vi "Module Init.vi"(8 "error in (no error)":errorcluster, 11 "DAQmxAO in":refnum<class "DAQmxAO.lvclass">) -> (0 "error out":errorcluster, 3 "DAQmxAO out":refnum<class "DAQmxAO.lvclass">)   [LabVIEW 2020, in "VolatusDAQ.lvlib" / "DAQmxAO.lvclass"]
uses:
  DAQmxAO.lvclass
  C:/dev/lv20CE/relink/lv-volatus/Volatus/Module/Module.lvclass
  Volatus/Message Registration.ctl
  VolatusData/DataProc Options.ctl
  DAQmxAO.lvclass/DAQmxAO.ctl
  Volatus/Module/Module.lvclass/Module.ctl
  Volatus/MessageQ/MessageQ.lvclass/MessageQ.ctl
  Volatus/Module/Self Q.vi
  Volatus/MessageQ/Send.vi
  VolatusDAQ.lvlib
  VolatusData/Data Processor Module/Data Processor Module.lvclass
  Volatus/Module/Module.lvclass
  Volatus/Volatus.lvlib
  VolatusData/VolatusData.lvlib
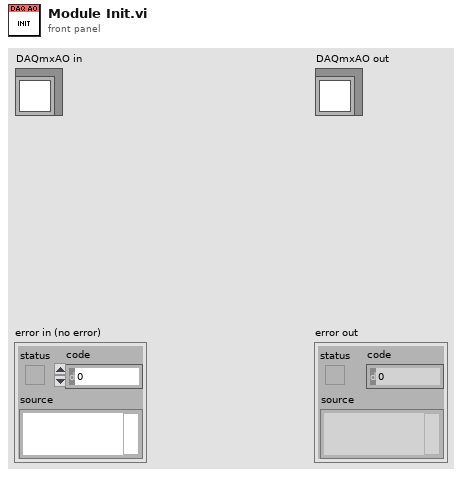
[diagram p1: front panel]
types:
  T1 = typedef "VolatusData.lvlib/DataProc Options.ctl" = cluster{"Ignore Scaling":bool}
  T2 = typedef "Volatus.lvlib/Message Registration.ctl" = cluster{"Message Type":string, "Message ID":string}
  T3 = typedef "VolatusDAQConfig.lvlib/Sampling Config.ctl" = cluster{"Rate":dbl, "Chunk Size":i32}
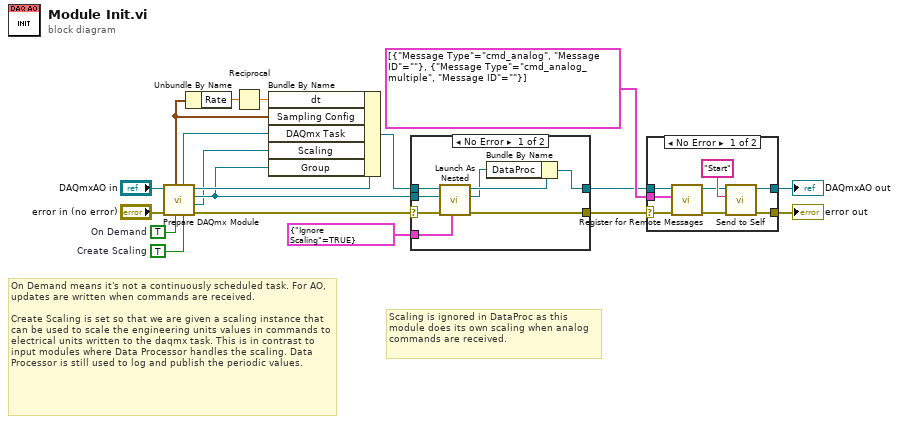
[diagram p0: block diagram]
diagram:
  w5 = TRUE  # On Demand
  w6 = TRUE  # Create Scaling
  # "Scaling is ignored in DataProc as this module does its own scaling when analog commands are received."
  # "On Demand means it's not a continuously scheduled task. For AO, updates are written when commands are received.\n\nCreate Scaling is set so that we are given a scaling instance that can be used to scale the engineering units values in commands to electrical units written to the daqmx task. This is in contrast to input modules where Data Processor handles the scaling. Data Processor is still used to log and publish the periodic values."
  n1 = call "Prepare DAQmx Module.vi"("Create Scaling (F)"=w6, "On Demand (F)"=w5, "error in (no error)"="error in (no error)", "Module in"="DAQmxAO in") -> ("error out"=w15:errorcluster, "Scaling"=w10:refnum<class "Scaling.lvclass">, "Group"=w13:refnum<class "Group.lvclass">, "Module out"=w17:refnum<class "DAQmxAO.lvclass">, "DAQmx Task"=w16:refnum<k21>, "Sampling Config"=w4:T3)  [unwired: 2 in]
  n2 = Unbundle By Name(w4) -> ("Rate"=w3:dbl)
  n3 = Reciprocal(x=w3) -> (1/x=w2:dbl)
  n4 = Bundle By Name(cluster=w17, "dt"=w2, "Sampling Config"=w4, "DAQmx Task"=w16, "Scaling"=w10, "Group"=w13) -> (w14:refnum<class "DAQmxAO.lvclass">)
  n5 = case shown="No Error" w15 {
    selector: w15 -> [w27 w28]
    tunnel: w14 -> [w26 w29]
    tunnel: w13 -> [w25 _]
    tunnel: [w24 w28] -> w7
    tunnel: [w21 w29] -> w8
    tunnel: T1 {"Ignore Scaling"=TRUE} ("DataProc Options") -> [w20 _]
    frame No Error {
      n6 = call "Launch As Nested.vi"("DataProc Options"=w20, "error in (no error)"=w27, "Group"=w25, "Parent in"=w26) -> ("error out"=w24:errorcluster, "MessageQ"=w22:refnum<class "MessageQ.lvclass">, "Parent out"=w23:refnum<class "DAQmxAO.lvclass">)  [unwired: 5 in]
      n7 = Bundle By Name(cluster=w23, "DataProc"=w22) -> (w21:refnum<class "DAQmxAO.lvclass">)
    }
    frame Error {
    }
  }
  n8 = case shown="No Error" w7 {
    selector: w7 -> [w32 w39]
    tunnel: [w37 w39] -> w11
    tunnel: w8 -> [w33 w38]
    tunnel: [w36 w38] -> w12
    tunnel: T2[] [{"Message Type"="cmd_analog", "Message ID"=""}, {"Message Type"="cmd_analog_multiple", "Message ID"=""}] ("Messages") -> [w34 _]
    frame No Error {
      n9 = call "Register for Remote Messages.vi"("error in (no error)"=w32, "Messages"=w34, "Module in"=w33) -> ("error out"=w30:errorcluster, "Module out"=w31:refnum<class "DAQmxAO.lvclass">)  [unwired: 7 in]
      n10 = call "Send to Self.vi"("error in (no error)"=w30, "Message ID"="Start", "Module in"=w31) -> ("error out"=w37:errorcluster, "Module out"=w36:refnum<class "DAQmxAO.lvclass">)  [unwired: 7 in]
    }
    frame Error {
    }
  }
  "error out" <- w11
  "DAQmxAO out" <- w12
